vi "Lookup_Table.vi"(0 "Y_Array":dbl[](array[numeric]) format="%.2f", 1 "x_in":dbl, 2 "X_Array":dbl[](array[numeric]) format="%.2f") -> (6 "y_out":dbl format="%.2f")   [LabVIEW 2019, in "ArgosLib.lvlib"]
uses:
  ArgosLib.lvlib
panel:
  # "Lookup_Table"
  # "This subsystem is a lookup table and will linerly interolate between points in the array"
  # "Tunning"
  # "Inputs"
  # "Outputs"
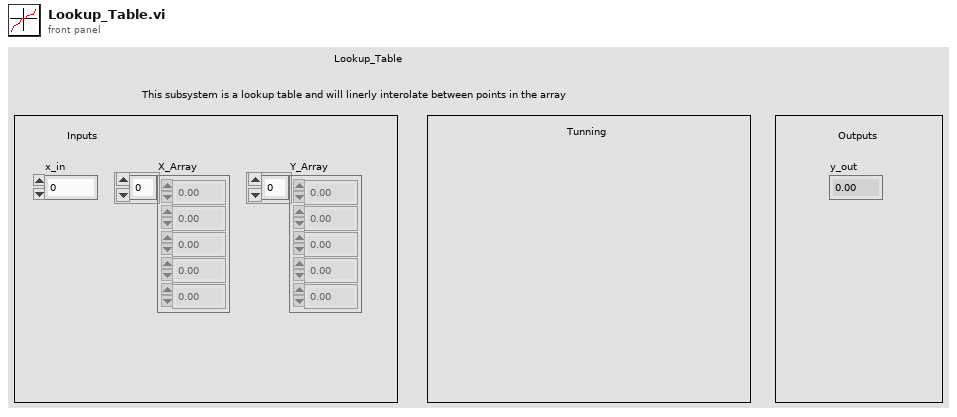
[diagram p1: front panel]
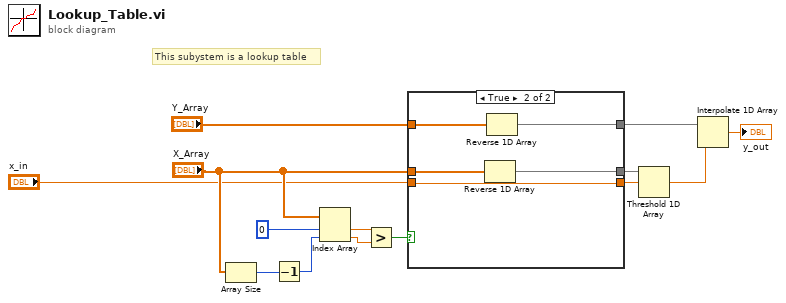
[diagram p0: block diagram]
diagram:
  # "This subystem is a lookup table"
  n1 = Array Size(array="X_Array") -> (size(s)=w1:i32)
  n2 = Decrement(x=w1) -> (x-1=w12:i32)
  n3 = Index Array(array="X_Array", index #1=0 ("index"), index #2=w12) -> (element #1=w10:dbl, element #2=w9:dbl)
  n4 = Greater?(x=w10, y=w9) -> (0:w8:bool)
  n5 = case shown="True" w8 {
    tunnel: "Y_Array" -> [w15 w22]
    tunnel: "X_Array" -> [w16 w21]
    tunnel: "x_in" -> [w17 w18]
    tunnel: [w17 w18] -> w4
    tunnel: [w16 w19] -> w3
    tunnel: [w15 w20] -> w2
    frame False {
    }
    frame True {
      n6 = Reverse 1D Array(array=w21) -> (reversed array=w19:dbl[])
      n7 = Reverse 1D Array(array=w22) -> (reversed array=w20:dbl[])
    }
  }
  n8 = Threshold 1D Array(2:w4, 3:w3) -> (0:w13:dbl)  [unwired: 1 in]
  n9 = Interpolate 1D Array(1:w13, 2:w2) -> (0:→"y_out":dbl)
